vi "PicoScope3000aSetupStreaming.vi"(0 "error in":errorcluster, 1 "Device Info":T2, 2 "handle in":i16, 3 "Acquisition Settings":T3={"Auto Stop"=FALSE, "Desired Sample Interval"=4, "Pre-trigger Samples"=0, "Post-trigger Samples"=1000, "Down-Sample Ratio"=1, "Down-Sample Mode"=0, "Time Units"=2} {"Time Units" items=["Nanoseconds (ns)"=2, "Microseconds (us)"=3, "Milliseconds (ms)"=4, "Seconds (s)"=5]; "Down-Sample Mode" items=["None"=0, "Aggregate"=1, "Decimate"=2, "Average"=4]}, 4 "Buffer and Transfer Settings":T1={"startIndex"=0, "Samples"=1000000, "Down Sample Ratio"=1, "Down-Sample Mode"=0} {"Down-Sample Mode" items=["None"=0, "Aggregate"=1, "Decimate"=2, "Average"=4]; "Down Sample Ratio" step=1; "Samples" format="%_6p"}, 5 "enabled array":i16[](array[numeric]), 6 "deviceIndex":u16, 10 "Pointers In":u64[][](array[numeric])) -> (11 "Pointer array":u64[][](array[numeric]), 14 "error out":errorcluster, 16 "handle out":i16, 17 "Sample Interval":u32, 19 "sampleIntervalTimeUnits":u32)   [LabVIEW 2016]
doc: "Set up the data buffers and calls RunStreaming to start the device streaming.\nData will be copied from the driver buffers into the corresponding application buffers using the wrapper dll."
uses:
  ps3000a.dll
  ps3000aWrap.dll
panel:
  # "Overview Buffer Size is the size of the temporary buffers used to\nstore data before returning it to the application."
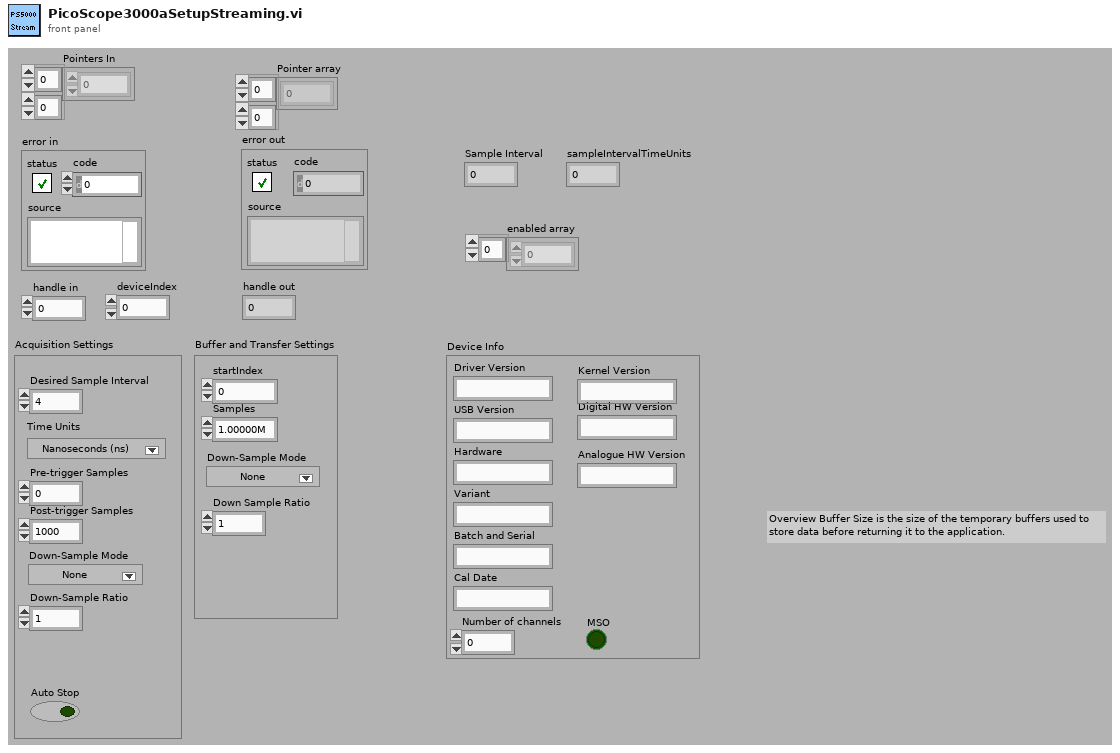
[diagram p1: front panel]
types:
  T1 = cluster{"startIndex":u64, "Samples":u64, "Down Sample Ratio":u64, "Down-Sample Mode":u32}
  T2 = cluster{"Driver Version":string, "USB Version":string, "Hardware":string, "Variant":string, "Batch and Serial":string, "Cal Date":string, "Kernel Version":string, "Digital HW Version":string, "Analogue HW Version":string, "MSO":bool, "Number of channels":i16}
  T3 = cluster{"Auto Stop":bool, "Desired Sample Interval":u32, "Pre-trigger Samples":u32, "Post-trigger Samples":u32, "Down-Sample Ratio":u32, "Down-Sample Mode":i32, "Time Units":u32}
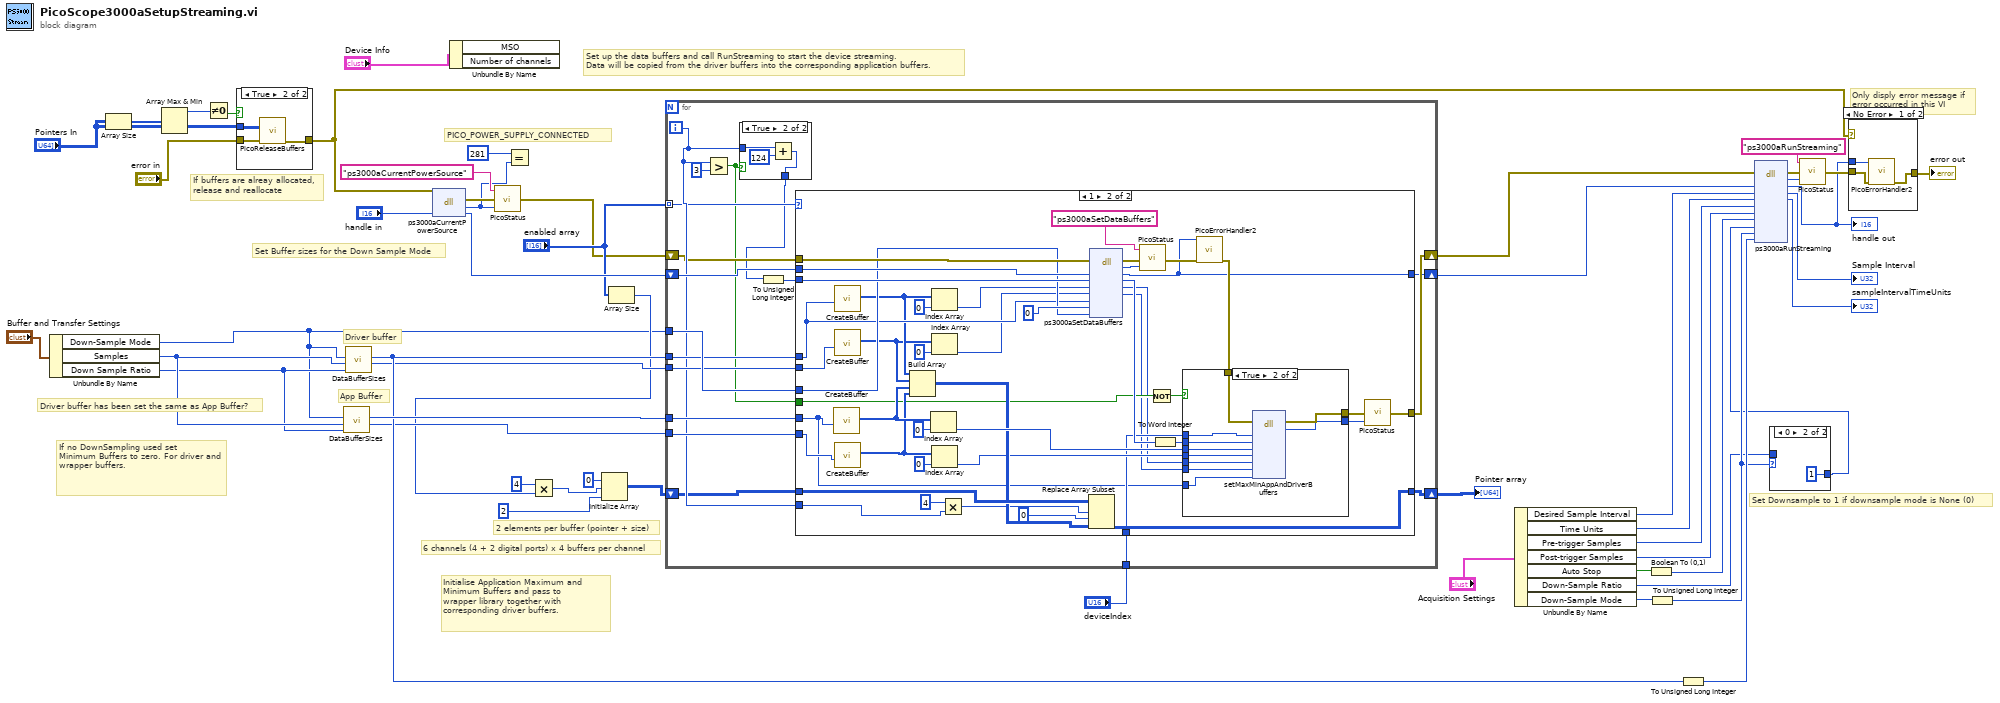
[diagram p0: block diagram]
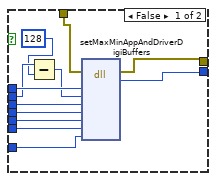
[diagram p6: hidden frame]
diagram:
  # "Set Downsample to 1 if downsample mode is None (0)"
  # "If buffers are alreay allocated,\nrelease and reallocate"
  # "2 elements per buffer (pointer + size)"
  # "6 channels (4 + 2 digital ports) x 4 buffers per channel"
  # "App Buffer"
  # "Driver buffer"
  # "Driver buffer has been set the same as App Buffer?"
  # "Set Buffer sizes for the Down Sample Mode"
  # "If no DownSampling used set \nMinimum Buffers to zero. For driver and wrapper buffers."
  # "PICO_POWER_SUPPLY_CONNECTED"
  # "Initialise Application Maximum and\nMinimum Buffers and pass to \nwrapper library together with corresponding driver buffers."
  # "Only disply error message if\nerror occurred in this VI"
  # "Set up the data buffers and call RunStreaming to start the device streaming.\nData will be copied from the driver buffers into the corresponding application buffers."
  n1 = Unbundle By Name("Buffer and Transfer Settings") -> ("Down-Sample Mode"=w6:u32, "Samples"=w31:u64, "Down Sample Ratio"=w30:u64)
  n2 = Array Size(array="Pointers In") -> (size(s)=w9:i32[])
  n3 = Array Max & Min(array=w9) -> (max value=w8:i32)  [unwired: 3 out]
  n4 = Not Equal To 0?(x=w8) -> (x != 0?=w16:bool)
  n5 = case shown="True" w16 {
    tunnel: "Pointers In" -> [_ w55]
    tunnel: "error in" -> [w54 w56]
    tunnel: [w54 w57] -> w13
    frame False {
    }
    frame True {
      n6 = call "PicoReleaseBuffers.vi"("error in (no error)"=w56, "Pointer array"=w55) -> ("error out"=w57:errorcluster)  [unwired: 9 in]
    }
  }
  n7 = call "DataBufferSizes.vi"("Down Sample Ratio"=w30, "Number of Samples"=w31, "Down-Sample Mode"=w6) -> ("min Buffer Size"=w26:i32, "Max Buffer Size"=w29:i32)  [unwired: 7 in]
  n8 = call "DataBufferSizes.vi"("Down Sample Ratio"=w30, "Number of Samples"=w31, "Down-Sample Mode"=w6) -> ("min Buffer Size"=w27:i32, "Max Buffer Size"=w28:i32)  [unwired: 7 in]
  n9 = dll-call lib="ps3000a.dll" fn="ps3000aCurrentPowerSource"(error in=w13, "handle"="handle in") -> (error out=w38:errorcluster, "PICO_STATUS"=w36:u32, "handle"=w34:i16)  [unwired: 2 in, 1 out]
  n10 = Unbundle By Name("Device Info") -> ()  [unwired: 2 out]
  n11 = call "PicoStatus.vi"("PICO STATUS"=w36, "error in"=w38, "source"="ps3000aCurrentPowerSource") -> ("error out"=w12:errorcluster)
  n12 = Equal?(x=u32 281, y=w36) -> ()  [unwired: 1 out]
  n13 = Array Size(array="enabled array") -> (size(s)=w20:i32)
  n14 = Multiply(x=4, y=w20) -> (x*y=w21:i32)
  n15 = Initialize Array(u64 0 ("element"), w21, 2 ("dimension size")) -> (w10:u64[][])
  n16 = for {
    tunnel: "enabled array" -> [w66] mode=indexing
    tunnel: w6 -> [w74]
    tunnel: w29 -> [w73]
    tunnel: w28 -> [w72]
    tunnel: w27 -> [w71]
    tunnel: w26 -> [w70]
    shift-right: [w65] -> w17
    shift-left: w12 -> [w64]
    shift-right: [w69] -> w25
    shift-left: w10 -> [w63]
    tunnel: "deviceIndex" -> [w60]
    shift-right: [w58] -> w1
    shift-left: w34 -> [w75]
    i -> [w67]
    n17 = Greater?(x=w67, y=3) -> (0:w59:bool)
    n18 = case shown="True" w59 {
      tunnel: [w76 w77] -> w61
      tunnel: w67 -> [w76 w79]
      frame False {
      }
      frame True {
        n19 = Add(x=w79, y=124) -> (x+y=w77:i32)
      }
    }
    n20 = To Unsigned Long Integer(number=w61) -> (unsigned 32bit integer=w62:u32)
    n21 = case shown="1" w66 {
      tunnel: w75 -> [w81 w126]
      tunnel: w64 -> [w80 w125]
      tunnel: w62 -> [_ w118]
      tunnel: w73 -> [_ w86]
      tunnel: w72 -> [_ w108]
      tunnel: w71 -> [_ w111]
      tunnel: w70 -> [_ w110]
      tunnel: w74 -> [_ w109]
      tunnel: w63 -> [w82 w102]
      tunnel: [w82 w101] -> w69
      tunnel: w67 -> [_ w98]
      tunnel: [w81 w85] -> w58
      tunnel: [w80 w94] -> w65
      tunnel: w60 -> [_ w89]
      tunnel: w59 -> [_ w87]
      frame 0, Default {
      }
      frame 1 {
        n22 = call "CreateBuffer.vi"("Buffer size"=w86) -> ("Pointer and BufferSize"=w104:u64[])  [unwired: 9 in, 1 out]
        n23 = call "CreateBuffer.vi"("Buffer size"=w108) -> ("Pointer and BufferSize"=w106:u64[])  [unwired: 9 in, 1 out]
        n24 = call "CreateBuffer.vi"("Buffer size"=w111) -> ("Pointer and BufferSize"=w105:u64[])  [unwired: 9 in, 1 out]
        n25 = call "CreateBuffer.vi"("Buffer size"=w110) -> ("Pointer and BufferSize"=w103:u64[])  [unwired: 9 in, 1 out]
        n26 = Build Array(w106, w105, w104, w103) -> (w97:u64[][])
        n27 = Index Array(array=w104, index=0) -> (element=w107:u64)
        n28 = Index Array(array=w106, index=0) -> (element=w100:u64)
        n29 = Index Array(array=w105, index=0) -> (element=w90:u64)
        n30 = Index Array(array=w103, index=0) -> (element=w91:u64)
        n31 = Multiply(x=4, y=w98) -> (x*y=w96:i32)
        n32 = Replace Array Subset(array=w102, new element=w97, index (row)=w96, index (col)=0 ("disabled index (row)")) -> (w101:u64[][])
        n33 = dll-call lib="ps3000a.dll" fn="ps3000aSetDataBuffers" ("ps3000.dll:_ps3000_open_unit@0")(error in=w125, "handle"=w126, "channel"=w118, "bufferMax"=w100, "bufferMin"=w90, "bufferLth"=w108, "segmentIndex"=u32 0, "downSampleRatioMode"=w109) -> (error out=w123:errorcluster, "PICO_STATUS"=w124:u32, "handle"=w85:i16, "channel"=w119:u32, "bufferMax"=w84:u64, "bufferMin"=w83:u64)  [unwired: 5 in, 1 out]
        n34 = call "PicoStatus.vi"("PICO STATUS"=w124, "error in"=w123, "source"="ps3000aSetDataBuffers") -> ("error out"=w93:errorcluster)
        n35 = Not(x=w87) -> (.not. x?=w88:bool)
        n36 = To Word Integer(number=w119) -> (16bit integer=w120:i16)
        n37 = call "PicoErrorHandler2.vi"("error in (no error)"=w93, "handle In"=w85) -> ("error out"=w92:errorcluster)  [unwired: 9 in]
        n38 = case shown="True" w88 {
          tunnel: w120 -> [w128 w148]
          tunnel: [w133 w147] -> w117
          tunnel: [w132 w146] -> w116
          tunnel: w107 -> [w137 w145]
          tunnel: w84 -> [w135 w144]
          tunnel: w92 -> [w138 w143]
          tunnel: w91 -> [w136 w142]
          tunnel: w83 -> [w134 w141]
          tunnel: w89 -> [w130 w140]
          tunnel: w86 -> [w131 w139]
          frame False {
            n39 = Subtract(x=w128, y=i16 128) -> (x-y=w129:i16)
            n40 = dll-call lib="ps3000aWrap.dll" fn="setMaxMinAppAndDriverDigiBuffers"(error in=w138, "deviceIndex"=w130, "digiport"=w129, "appMaxDigiBuffer"=w137, "appMinDigiBuffer"=w136, "driverMaxDigiBuffer"=w135, "driverMinDigiBuffer"=w134, "bufferLength"=w131) -> (error out=w133:errorcluster, "PICO STATUS"=w132:u32)  [unwired: 9 in, 1 out]
          }
          frame True {
            n41 = dll-call lib="ps3000aWrap.dll" fn="setMaxMinAppAndDriverBuffers"(error in=w143, "deviceIndex"=w140, "channel"=w148, "appMaxBuffer"=w145, "appMinBuffer"=w142, "driverMaxBuffer"=w144, "driverMinBuffer"=w141, "bufferLength"=w139) -> (error out=w147:errorcluster, "status"=w146:u32)  [unwired: 9 in, 1 out]
          }
        }
        n42 = call "PicoStatus.vi"("PICO STATUS"=w116, "error in"=w117) -> ("error out"=w94:errorcluster)  [unwired: 1 in]
      }
    }
  }
  "Pointer array" <- w25
  n43 = Unbundle By Name("Acquisition Settings") -> ("Desired Sample Interval"=w46:u32, "Time Units"=w40:u32, "Pre-trigger Samples"=w45:u32, "Post-trigger Samples"=w44:u32, "Auto Stop"=w43:bool, "Down-Sample Ratio"=w4:u32, "Down-Sample Mode"=w41:i32)
  n44 = Boolean To (0,1)(Boolean=w43) -> (0, 1=w47:i16)
  n45 = To Unsigned Long Integer(number=w41) -> (unsigned 32bit integer=w5:u32)
  n46 = To Unsigned Long Integer(number=w28) -> (unsigned 32bit integer=w7:u32)
  n47 = case shown="0" w5 {
    tunnel: [w149 u32 1 ("Down-Sample Ratio")] -> w3
    tunnel: w4 -> [w149 _]
    frame Default {
    }
    frame 0 {
    }
  }
  n48 = dll-call lib="ps3000a.dll" fn="ps3000aRunStreaming" ("ps5000a.dll:_ps3000_open_unit@0")(error in=w17, "handle"=w1, "sampleInterval"=w46, "sampleIntervalTimeUnits"=w40, "maxPreTriggerSamples"=w45, "maxPostTriggerSamples"=w44, "autoStop"=w47, "downSampleRatio"=w3, "downSampleRatioMode"=w5, "overviewBufferSize"=w7) -> (error out=w51:errorcluster, "PICO_STATUS"=w52:u32, "handle"=w11:i16, "sampleInterval"=→"Sample Interval":u32, "sampleIntervalTimeUnits"=→"sampleIntervalTimeUnits":u32)  [unwired: 8 in, 1 out]
  "handle out" <- w11
  n49 = call "PicoStatus.vi"("PICO STATUS"=w52, "error in"=w51, "source"="ps3000aRunStreaming") -> ("error out"=w49:errorcluster)
  n50 = case shown="No Error" w13 {
    tunnel: [w152 w154] -> w53
    tunnel: w49 -> [w153 w154]
    tunnel: w11 -> [w151 _]
    frame No Error {
      n51 = call "PicoErrorHandler2.vi"("error in (no error)"=w153, "handle In"=w151) -> ("error out"=w152:errorcluster)  [unwired: 9 in]
    }
    frame Error {
    }
  }
  "error out" <- w53
